vi "UpdateVIIcon.vi"(8 "error in (no error)":errorcluster, 10 "Method Name":string, 11 "VI in":refnum<vi>) -> (0 "error out":errorcluster, 3 "VI out":refnum<vi>)   [LabVIEW 2019, in "gRPC Template Creation Utility.lvlib"]
uses:
  gRPC Template Creation Utility.lvlib
  <vilib>/LabVIEW Icon API/API_Text.ctl
  <vilib>/LabVIEW Icon API/LabVIEW Icon API.lvlib
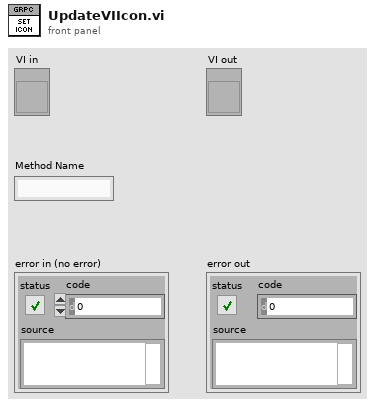
[diagram p1: front panel]
types:
  T1 = typedef "LabVIEW Icon API.lvlib/API_Text.ctl" = cluster{"Line 1 text":string, "Line 2 text":string, "Line 3 text":string, "Line 4 text":string}
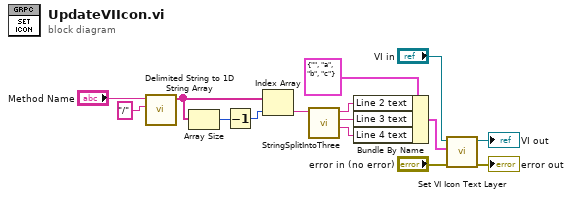
[diagram p0: block diagram]
diagram:
  n1 = call <vilib>:"Delimited String to 1D String Array.vi"("delimiter"="/", "delimited string"="Method Name") -> ("string array"=w6:string[])  [unwired: 9 in]
  n2 = Array Size(array=w6) -> (size(s)=w5:i32)
  n3 = Decrement(x=w5) -> (x-1=w4:i32)
  n4 = Index Array(array=w6, index=w4) -> (element=w3:string)
  n5 = call "StringSplitIntoThree.vi"("String"=w3) -> ("Line 3"=w9:string, "Line 2"=w10:string, "Line 1"=w11:string)  [unwired: 8 in]
  n6 = Bundle By Name(cluster=T1 {"Line 1 text"="", "Line 2 text"="a", "Line 3 text"="b", "Line 4 text"="c"} ("Text"), "Line 2 text"=w11, "Line 3 text"=w10, "Line 4 text"=w9) -> (w12:T1)
  n7 = call "Set VI Icon Text Layer.vi"("error in (no error)"="error in (no error)", "Text"=w12, "VI in"="VI in") -> ("error out"=→"error out":errorcluster, "VI out"=→"VI out":refnum<vi>)  [unwired: 7 in]
